vi "Room_Grid.vi"(0 "State":T2={"Tick"=0, "Phase"=0, "PhaseTicks"=0, "Level"=1, "Room"=0, "X10"=0, "Y10"=0, "VY10"=0, "Mode"=0, "Facing"=0, "Run"=0, "Vert"=0, "StandY"=0, "EntryX10"=0, "EntryY10"=0, "EntryMode"=0, "Lives"=4, "Score"=0, "NextLife"=10000, "KeyR"=0, "KeyB"=0, "KeyY"=0, "Torch"=FALSE, "FloorPhase"=0, "Dead"=FALSE, "LevelStart"=FALSE, "Quit"=FALSE, "Sound"=0, "Seed"=12345, "DemoStep"=0, "Tiles"=[], "World"=[], "Enemies"=[], "Highscores"=[], "Name"=[0, 0, 0], "Cursor"=0}, 5 "Memory":T1={"RoomKey"=-1, "Key"=-1, "NameKey"=-1, "Lit"=[], "Dim"=[], "Dark"=[], "Comp"=[], "Template"={"image type"=0, "image depth"=0, "image"=[], "mask"=[], "colors"=[], "Rectangle"={"left"=0, "top"=0, "right"=0, "bottom"=0}}, "CX"=-1, "CY"=-1, "X1"=0, "Y1"=0, "X2"=0, "Y2"=0, "Prev"=[], "HudKey"=-1, "HudScore"=-1, "HudTime"=-1, "Full"=[]}, 11 "error in":errorcluster) -> (4 "Grid":u8[][](array[numeric]), 6 "Memory out":T1={"RoomKey"=-1, "Key"=-1, "NameKey"=-1, "Lit"=[], "Dim"=[], "Dark"=[], "Comp"=[], "Template"={"image type"=0, "image depth"=0, "image"=[], "mask"=[], "colors"=[], "Rectangle"={"left"=0, "top"=0, "right"=0, "bottom"=0}}, "CX"=-1, "CY"=-1, "X1"=0, "Y1"=0, "X2"=0, "Y2"=0, "Prev"=[], "HudKey"=-1, "HudScore"=-1, "HudTime"=-1, "Full"=[]}, 8 "Dark":bool, 15 "error out":errorcluster)   [LabVIEW 2020, in "GH_Render.lvlib"]
doc: "The room raster of this frame: loads the three room pictures (lit, dim, dark) on a new room or level and keeps them in Memory; in a dark room (deep enough, no torch, not on the title, not the treasure room) the composite whose light circle around Claude Light_Update moves only when Claude changes the tile. Grid = composite when Dark, else the lit picture."
uses:
  GH_Render.lvlib
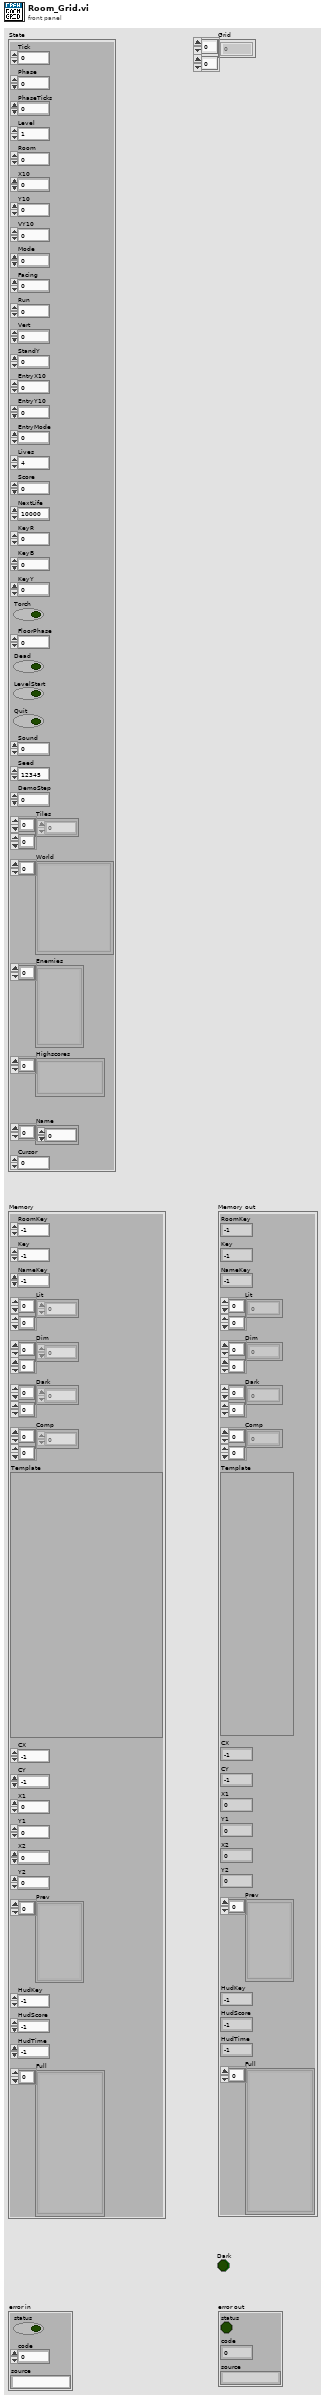
[diagram p1: front panel]
types:
  T1 = cluster{"RoomKey":i32, "Key":i32, "NameKey":i32, "Lit":u8[][], "Dim":u8[][], "Dark":u8[][], "Comp":u8[][], "Template":cluster{"image type":i32, "image depth":i32, "image":u8[], "mask":u8[], "colors":u32[], "Rectangle":cluster{"left":i16, "top":i16, "right":i16, "bottom":i16}}, "CX":i32, "CY":i32, "X1":i32, "Y1":i32, "X2":i32, "Y2":i32, "Prev":cluster{"Kind":i32, "X10":i32, "Y10":i32, "Dir":i32, "Mode":i32}[], "HudKey":i32, "HudScore":i32, "HudTime":i32, "Full":cluster{"image type":i32, "image depth":i32, "image":u8[], "mask":u8[], "colors":u32[], "Rectangle":cluster{"left":i16, "top":i16, "right":i16, "bottom":i16}}[]}
  T2 = cluster{"Tick":u32, "Phase":i32, "PhaseTicks":i32, "Level":i32, "Room":i32, "X10":i32, "Y10":i32, "VY10":i32, "Mode":i32, "Facing":i32, "Run":i32, "Vert":i32, "StandY":i32, "EntryX10":i32, "EntryY10":i32, "EntryMode":i32, "Lives":i32, "Score":i32, "NextLife":i32, "KeyR":i32, "KeyB":i32, "KeyY":i32, "Torch":bool, "FloorPhase":i32, "Dead":bool, "LevelStart":bool, "Quit":bool, "Sound":i32, "Seed":u32, "DemoStep":i32, "Tiles":u8[][], "World":cluster{"ID":string, "Depth":i32, "Column":i32, "Tiles":u8[][]}[], "Enemies":cluster{"Kind":i32, "X10":i32, "Y10":i32, "Dir":i32, "Mode":i32}[], "Highscores":cluster{"Score":i32, "Name":string}[], "Name":i32[], "Cursor":i32}
  T3 = cluster{"ID":string, "Depth":i32, "Column":i32, "Tiles":u8[][]}[]
  T4 = cluster{"ID":string, "Depth":i32, "Column":i32, "Tiles":u8[][]}
  T5 = cluster{"image type":i32, "image depth":i32, "image":u8[], "mask":u8[], "colors":u32[], "Rectangle":cluster{"left":i16, "top":i16, "right":i16, "bottom":i16}}
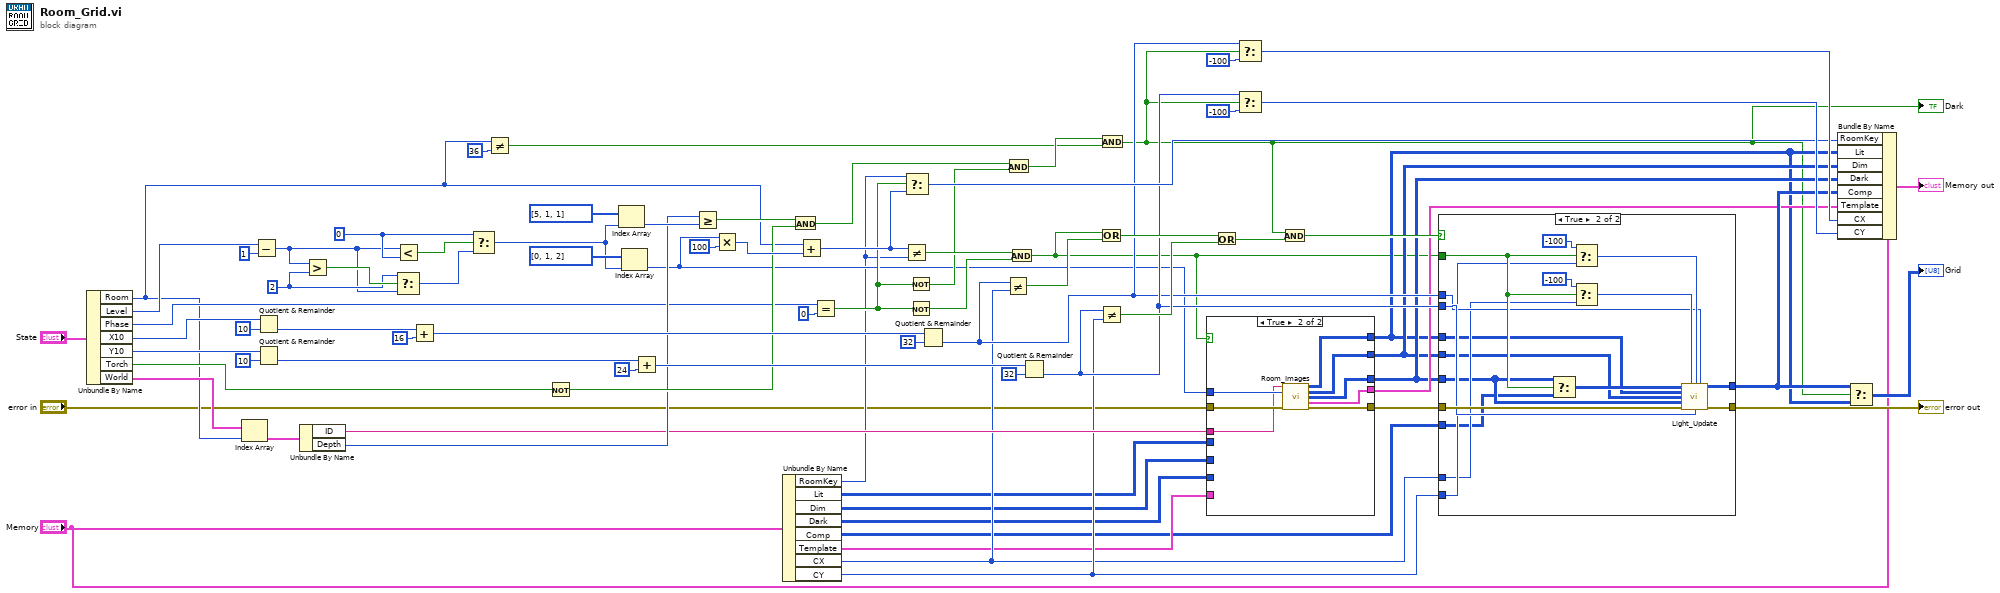
[diagram p0: block diagram]
diagram:
  w22 = 2
  w21 = 0
  n1 = Unbundle By Name("State") -> ("Room"=w4:i32, "Level"=w5:i32, "Phase"=w6:i32, "X10"=w7:i32, "Y10"=w8:i32, "Torch"=w9:bool, "World"=w10:T3)
  n2 = Index Array(array=w10, index=w4) -> (element=w29:T4)
  n3 = Subtract(x=w5, y=1) -> (x-y=w20:i32)
  n4 = Quotient & Remainder(x=w7, y=10) -> (floor(x/y)=w56:i32)  [unwired: 1 out]
  n5 = Quotient & Remainder(x=w8, y=10) -> (floor(x/y)=w58:i32)  [unwired: 1 out]
  n6 = Unbundle By Name(w29) -> ("ID"=w30:string, "Depth"=w31:i32)
  n7 = Greater?(x=w20, y=w22) -> (0:w24:bool)
  n8 = Less?(x=w20, y=w21) -> (x < y?=w23:bool)
  n9 = Select(t=w22, s=w24, f=w20) -> (s? t:f=w25:i32)
  n10 = Add(x=w56, y=16) -> (x+y=w60:i32)
  n11 = Select(t=w21, s=w23, f=w25) -> (s? t:f=w26:i32)
  n12 = Not Equal?(x=w4, y=36) -> (x != y?=w40:bool)
  n13 = Not(x=w9) -> (.not. x?=w37:bool)
  n14 = Index Array(array=i32[] [5, 1, 1] ("Dark from"), index=w26) -> (element=w35:i32)
  n15 = Index Array(array=i32[] [0, 1, 2] ("Theme"), index=w26) -> (element=w28:i32)
  n16 = Add(x=w58, y=24) -> (x+y=w64:i32)
  n17 = Greater Or Equal?(x=w31, y=w35) -> (x >= y?=w36:bool)
  n18 = Multiply(x=w28, y=100) -> (x*y=w45:i32)
  n19 = Unbundle By Name("Memory") -> ("RoomKey"=w11:i32, "Lit"=w12:u8[][], "Dim"=w13:u8[][], "Dark"=w14:u8[][], "Comp"=w15:u8[][], "Template"=w16:T5, "CX"=w17:i32, "CY"=w18:i32)
  n20 = And(x=w36, y=w37) -> (x .and. y?=w41:bool)
  n21 = Add(x=w4, y=w45) -> (x+y=w46:i32)
  n22 = Equal?(x=w6, y=0) -> (x = y?=w33:bool)
  n23 = Select(t=w11, s=w33, f=w46) -> (s? t:f=w75:i32)
  n24 = Not Equal?(x=w46, y=w11) -> (x != y?=w47:bool)
  n25 = Not(x=w33) -> (.not. x?=w38:bool)
  n26 = Not(x=w33) -> (.not. x?=w48:bool)
  n27 = Quotient & Remainder(x=w60, y=32) -> (floor(x/y)=w62:i32)  [unwired: 1 out]
  n28 = Not Equal?(x=w62, y=w17) -> (x != y?=w67:bool)
  n29 = And(x=w41, y=w38) -> (x .and. y?=w42:bool)
  n30 = And(x=w47, y=w48) -> (x .and. y?=w49:bool)
  n31 = Quotient & Remainder(x=w64, y=32) -> (floor(x/y)=w66:i32)  [unwired: 1 out]
  n32 = Or(x=w49, y=w67) -> (x .or. y?=w69:bool)
  n33 = Not Equal?(x=w66, y=w18) -> (x != y?=w68:bool)
  n34 = And(x=w42, y=w40) -> (x .and. y?=w43:bool)
  "Dark" <- w43
  n35 = case shown="True" w49 {
    tunnel: "error in" -> [w85 w88]
    tunnel: w12 -> [w81 _]
    tunnel: w13 -> [w82 _]
    tunnel: w14 -> [w83 _]
    tunnel: w16 -> [w84 _]
    tunnel: w30 -> [_ w86]
    tunnel: w28 -> [_ w87]
    tunnel: [w81 w89] -> w50
    tunnel: [w82 w90] -> w51
    tunnel: [w83 w91] -> w52
    tunnel: [w84 w92] -> w53
    tunnel: [w85 w93] -> w54
    frame False {
    }
    frame True {
      n36 = call "Room_Images.vi"("Room ID"=w86, "Theme"=w87, "error in"=w88) -> ("Lit"=w89:u8[][], "Dim"=w90:u8[][], "Dark"=w91:u8[][], "Template"=w92:T5, "error out"=w93:errorcluster)  [unwired: 8 in]
    }
  }
  n37 = Or(x=w69, y=w68) -> (x .or. y?=w70:bool)
  n38 = Select(t=w62, s=w43, f=-100) -> (s? t:f=w77:i32)
  n39 = Select(t=w66, s=w43, f=-100) -> (s? t:f=w79:i32)
  n40 = And(x=w43, y=w70) -> (x .and. y?=w71:bool)
  n41 = case shown="True" w71 {
    tunnel: w15 -> [w94 w96]
    tunnel: w17 -> [_ w100]
    tunnel: w18 -> [_ w101]
    tunnel: w62 -> [_ w102]
    tunnel: w66 -> [_ w103]
    tunnel: w50 -> [_ w97]
    tunnel: w51 -> [_ w98]
    tunnel: w52 -> [_ w99]
    tunnel: w54 -> [w95 w104]
    tunnel: w49 -> [_ w105]
    tunnel: [w94 w111] -> w72
    tunnel: [w95 w112] -> w73
    frame False {
    }
    frame True {
      n42 = Select(t=w99, s=w105, f=w96) -> (s? t:f=w106:u8[][])
      n43 = Select(t=-100, s=w105, f=w101) -> (s? t:f=w110:i32)
      n44 = Select(t=-100, s=w105, f=w100) -> (s? t:f=w108:i32)
      n45 = call "Light_Update.vi"("Comp"=w106, "Old CX"=w108, "Old CY"=w110, "CX"=w102, "Lit"=w97, "Dim"=w98, "Dark"=w99, "error in"=w104, "CY"=w103) -> ("Comp out"=w111:u8[][], "error out"=w112:errorcluster)  [unwired: 4 in, 1 out]
    }
  }
  "error out" <- w73
  n46 = Bundle By Name(cluster="Memory", "RoomKey"=w75, "Lit"=w50, "Dim"=w51, "Dark"=w52, "Comp"=w72, "Template"=w53, "CX"=w77, "CY"=w79) -> (→"Memory out":T1)
  n47 = Select(t=w72, s=w43, f=w50) -> (s? t:f=→"Grid":u8[][])
